vi "PeriodicFilter-Append Filtered Status.vi"(6 "Filtered Status":string[](array[string]), 11 "String Cache In":string) -> (3 "String Cache Out":string)   [LabVIEW 2017, in "Communicable State Machine.lvlib"]
uses:
  Communicable State Machine.lvlib
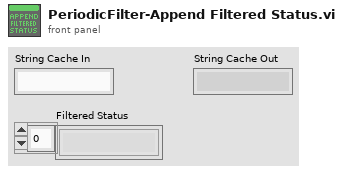
[diagram p1: front panel]
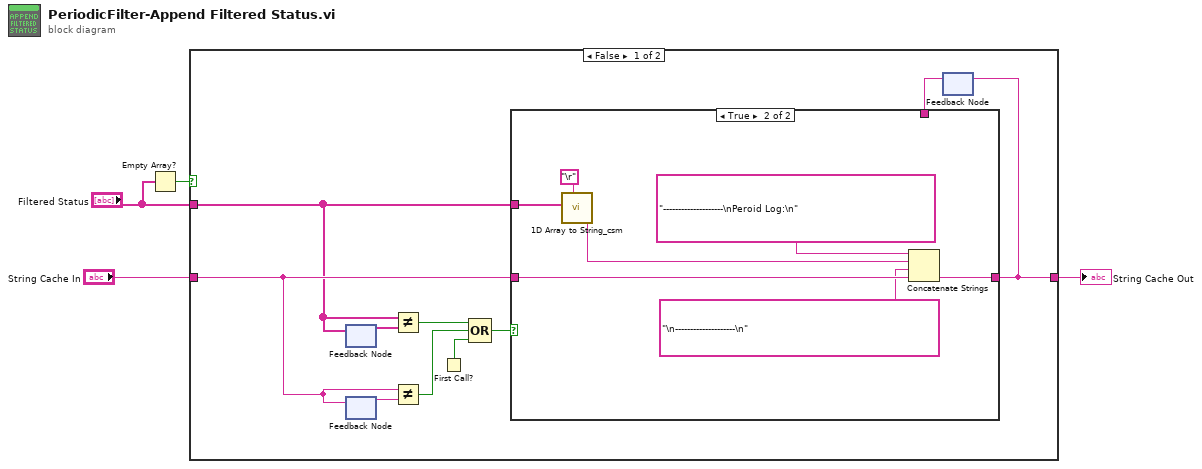
[diagram p0: block diagram]
diagram:
  n1 = Empty Array?(array="Filtered Status") -> (empty?=w4:bool)
  n2 = case shown="False" w4 {
    tunnel: "String Cache In" -> [w9 w23]
    tunnel: [w14 w23] -> w2
    tunnel: "Filtered Status" -> [w5 _]
    frame False {
      n3 = feedback #1() -> (w8:string[])  [unwired: 1 in]
      n4 = feedback-in #1(w5) -> ()
      n5 = feedback #2() -> (w10:string)  [unwired: 1 in]
      n6 = feedback-in #2(w9) -> ()
      n7 = Not Equal?(x=w5, y=w8) -> (x != y?=w7:bool)
      n8 = Not Equal?(x=w9, y=w10) -> (x != y?=w11:bool)
      n9 = First Call?() -> (First Call?: T/F=w12:bool)
      n10 = Compound Arithmetic op=OR(w7, w11, w12) -> (w6:bool)
      n11 = feedback #3() -> (w13:string)  [unwired: 1 in]
      n12 = case shown="True" w6 {
        tunnel: [w15 w22] -> w14
        tunnel: w5 -> [_ w19]
        tunnel: w9 -> [_ w21]
        tunnel: w13 -> [w15 _]
        frame False {
        }
        frame True {
          n13 = call "1D Array to String_csm.vi"("delimiter (Tab)"="\r" ("Carriage Return Constant"), "Array of Strings"=w19) -> ("delimited string"=w18:string)  [unwired: 9 in]
          n14 = Concatenate Strings("--------------------\nPeroid Log:\n" ("string"), w18, "\n--------------------\n" ("string"), w21) -> (w22:string)
        }
      }
      n15 = feedback-in #3(w14) -> ()
    }
    frame True {
    }
  }
  "String Cache Out" <- w2
